vi "PLC_Close.vi"(8 "error in (no error)":errorcluster, 11 "PLC Conn":refnum<visa-resource-name>) -> (0 "error out":errorcluster)   [LabVIEW 2018]
doc: "Use this template to build a VI to use as a subVI."
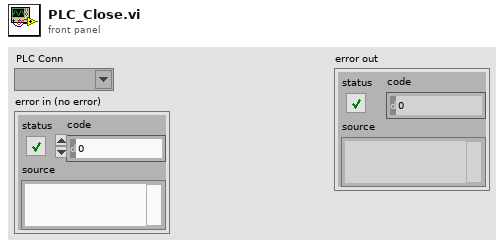
[diagram p1: front panel]
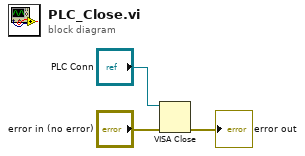
[diagram p0: block diagram]
diagram:
  n1 = VISA Close(VISA resource name="PLC Conn", error in (no error)="error in (no error)") -> (error out=→"error out":errorcluster)
